vi "SeqEditor_Global.vi"() -> ()   [LabVIEW 2017, in "NLTest.lvclass"]
uses:
  NLTest.lvclass
panel:
  in  "Step集选择行":i32
  in  "Param集单击值列？":bool
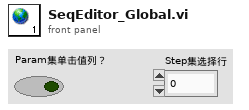
[diagram p1: front panel]
diagram:
